vi "Trigger Replay Metadata.vi"(8 "error in":errorcluster, 10 "Load UserEvents (Reply Payload)":T1) -> (0 "error out":errorcluster)   [LabVIEW 2026, in "Replay.lvlib"]
doc: "_____\nCreated using DQMH Framework: Event Scripter 7.1.2.1547."
uses:
  Replay.lvlib
  Load UserEvents (Reply Payload)--cluster.ctl
  Trigger Replay Metadata Argument--cluster.ctl
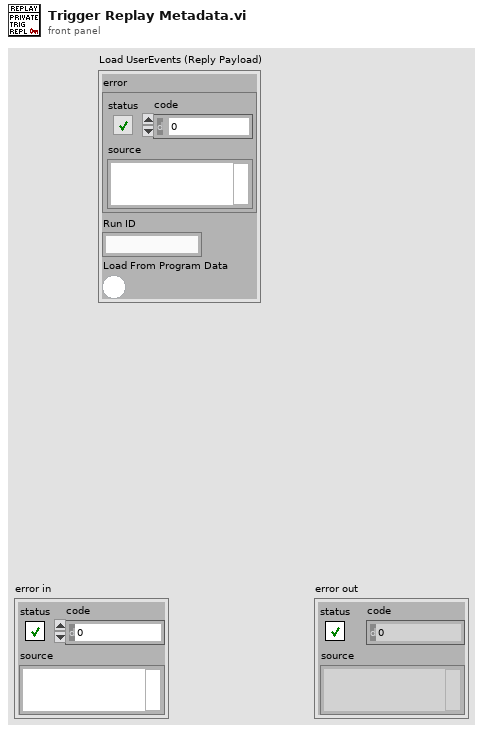
[diagram p1: front panel]
types:
  T1 = typedef "Replay.lvlib/Load UserEvents (Reply Payload)--cluster.ctl" = cluster{"error":errorcluster, "Run ID":string, "Load From Program Data":bool}
  T2 = typedef "Replay.lvlib/Trigger Replay Metadata Argument--cluster.ctl" = cluster{"Load UserEvents (Reply Payload)":T1}
  T3 = typedef "Replay.lvlib/Request Events--cluster.ctl" = cluster{"Stop Module":refnum<user-event>, "Show Panel":refnum<user-event>, "Hide Panel":refnum<user-event>, "Get Module Execution Status":refnum<user-event>, "Show Diagram":refnum<user-event>, "Set Run ID to Replay":refnum<user-event>, "Load UserEvents":refnum<user-event>, "Private.Trigger Replay Metadata":refnum<user-event>}
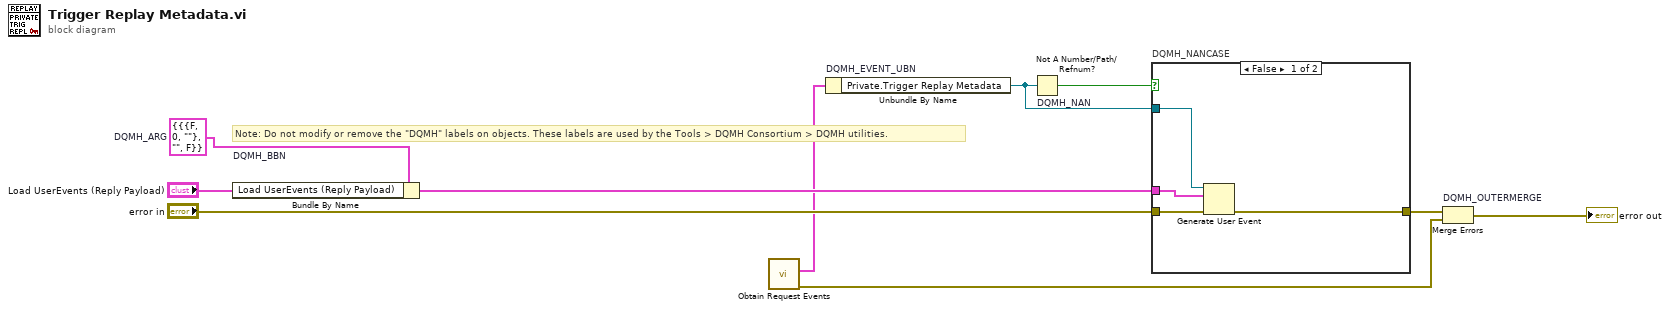
[diagram p0: block diagram]
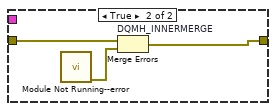
[diagram p2: hidden frame]
diagram:
  w4 = T2 {"Load UserEvents (Reply Payload)"={"error"={"status"=FALSE, "code"=0, "source"=""}, "Run ID"="", "Load From Program Data"=FALSE}}  # DQMH_ARG
  # "Note: Do not modify or remove the \"DQMH\" labels on objects. These labels are used by the Tools > DQMH Consortium > DQMH utilities."
  n1 = Bundle By Name "DQMH_BBN"(cluster=w4, "Load UserEvents (Reply Payload)"="Load UserEvents (Reply Payload)") -> (w8:T2)
  n2 = call "Obtain Request Events.vi"() -> ("error out"=w2:errorcluster, "Replay Request Events"=w1:T3)  [unwired: 10 in]
  n3 = Unbundle By Name "DQMH_EVENT_UBN"(w1) -> ("Private.Trigger Replay Metadata"=w6:refnum<user-event>)
  n4 = Not A Number/Path/Refnum? "DQMH_NAN"(number/path/refnum=w6) -> (NaN/Path/Refnum?=w7:bool)
  n5 = case "DQMH_NANCASE" shown="False" w7 {
    tunnel: "error in" -> [w14 w17]
    tunnel: [w13 w16] -> w5
    tunnel: w6 -> [w12 _]
    tunnel: w8 -> [w11 _]
    frame False {
      n6 = Generate User Event(user event=w12, event data cluster=w11, error in=w14) -> (error out=w13:errorcluster)  [unwired: 1 in, 1 out]
    }
    frame True {
      n7 = call "Module Not Running--error.vi"() -> ("error out"=w15:errorcluster)  [unwired: 11 in]
      n8 = Merge Errors "DQMH_INNERMERGE"(w17, w15) -> (w16:errorcluster)
    }
  }
  n9 = Merge Errors "DQMH_OUTERMERGE"(w5, w2) -> (→"error out":errorcluster)
